vi "Handle Messages.vi"(8 "error in (no error)":errorcluster, 9 "Message Data":variant, 10 "Message":string, 11 "Mock Rig Process In":refnum<class "Mock Process.lvclass">) -> (0 "error out":errorcluster, 3 "Mock Rig Process Out":refnum<class "Mock Process.lvclass">)   [LabVIEW 2020, in "Mock Process.lvclass"]
uses:
  Mock Process.lvclass
  C:/git/astemes-triarc-framework/source/Framework/Process/Process.lvclass
  C:/git/astemes-triarc-framework/source/Framework/Helper Loop/Helper Loop.lvclass
  Mock Process.lvclass/Mock Process.ctl
  Framework/Process/Process.lvclass/Process.ctl
  Framework/Process/Public/Lifecycle/Get Lifecycle State.vi
  Framework/Process/Private/SubVIs/Handle Debug Data.vi
  <vilib>/Utility/error.llb/Clear Errors.vi
  Framework/Logging/Log Debug.vi
  <vilib>/AdvancedString/1D String Array to Delimited String.vi
  <vilib>/Utility/High Resolution Relative Seconds.vi
  Framework/Process/Process.lvclass
  C:/git/astemes-triarc-framework/source/Framework/Logging/Logging.lvclass
  <vilib>/Utility/error.llb/Error Cluster From Error Code.vi
  Framework/Process/Public/Read Name.vi
  <vilib>/ErrorRing/Error Ring.xnode
  Framework/Callback/Callback.lvclass
  Framework/Logging/Logging.lvclass
  Framework/Helper Loop/Helper Loop.lvclass
  C:/git/astemes-triarc-framework/source/Framework/Base/Base.lvclass
  C:/git/astemes-triarc-framework/source/Framework/Configuration File/Configuration File.lvclass
  C:/git/astemes-triarc-framework/source/Framework/Configuration/Configuration.lvclass
  C:/git/astemes-triarc-framework/source/Framework/Error Handler Interface/Error Handler Interface.lvclass
  C:/git/astemes-triarc-framework/source/Framework Test Suite/Mock Process/Mock Process.lvclass
  C:/git/astemes-triarc-framework/source/Framework/Async Handler/Async Handler.lvclass
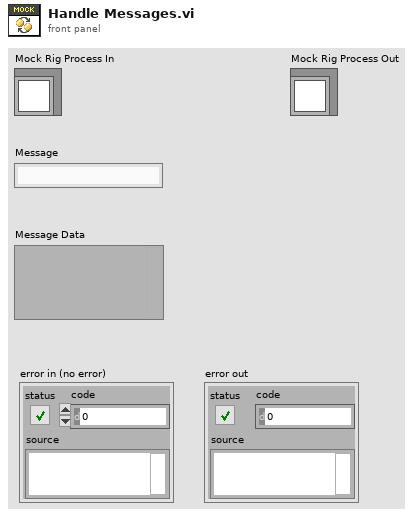
[diagram p1: front panel]
types:
  T1 = cluster{"Message":string, "Message Data":variant}
  T2 = cluster{"Request Message":string, "Request Message Data":variant}
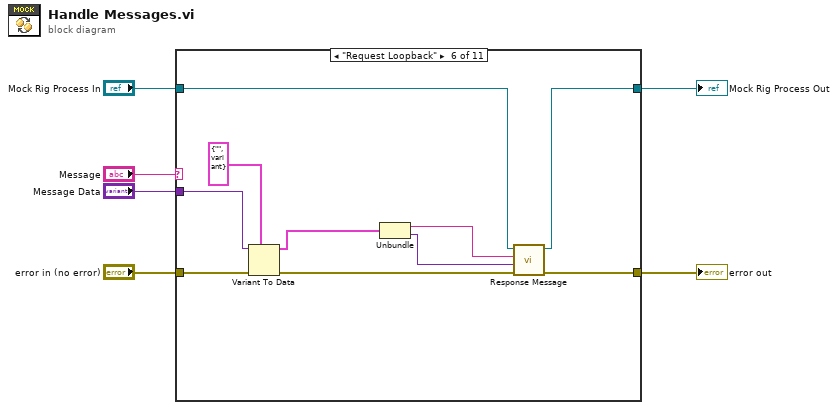
[diagram p0: block diagram]
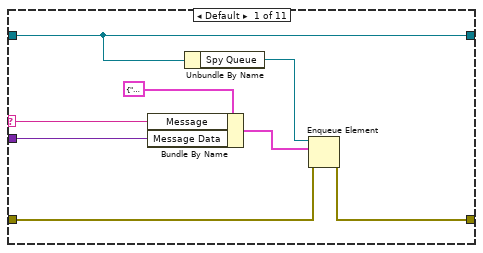
[diagram p2: hidden frame]
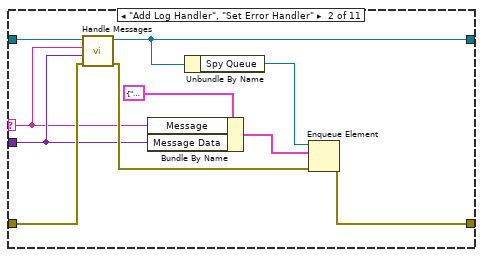
[diagram p3: hidden frame]
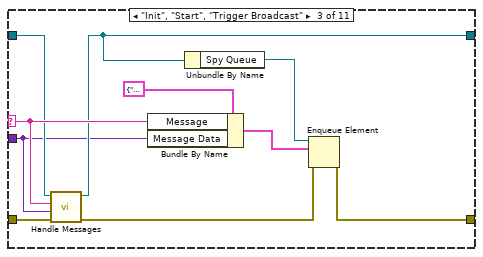
[diagram p4: hidden frame]
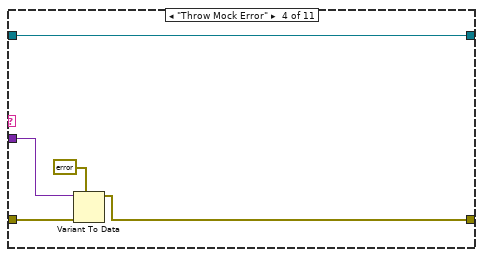
[diagram p5: hidden frame]
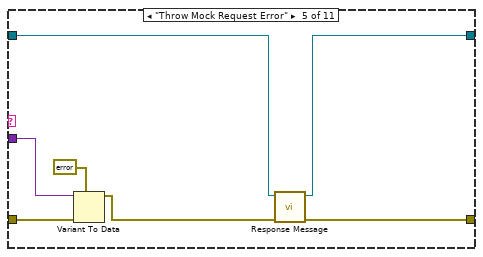
[diagram p6: hidden frame]
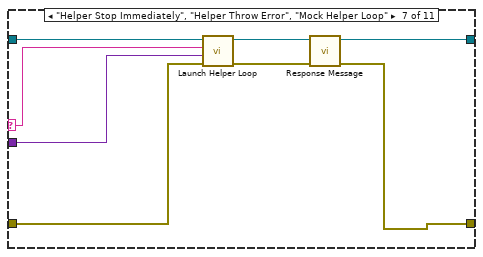
[diagram p7: hidden frame]
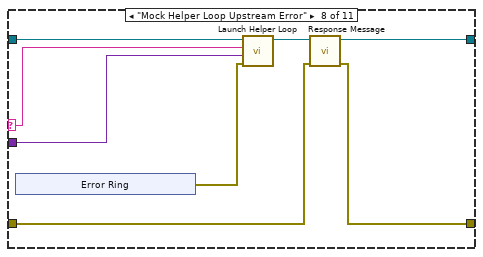
[diagram p8: hidden frame]
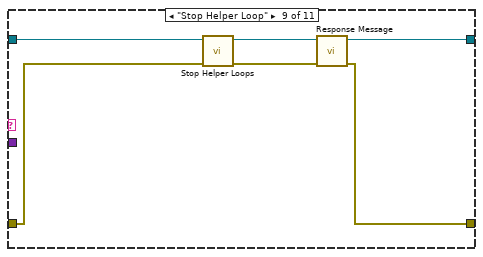
[diagram p9: hidden frame]
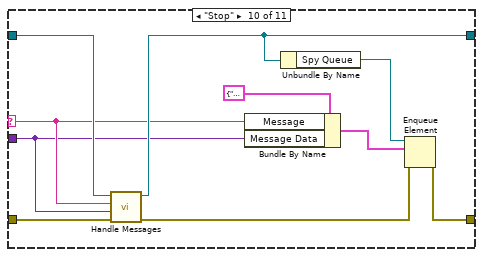
[diagram p10: hidden frame]
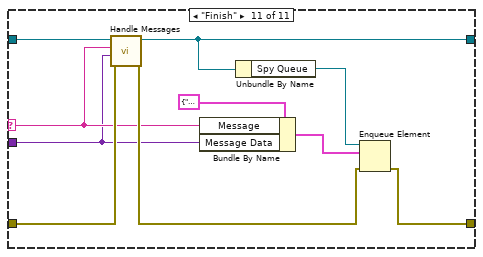
[diagram p11: hidden frame]
diagram:
  n1 = case shown="\"Request Loopback\"" "Message" {
    selector: "Message" -> [w10 w15 w28 _ _ _ w61 w71 _ w84 w94]
    tunnel: [w8 w20 w30 w35 w42 w55 w59 w69 w79 w89 w95] -> w6
    tunnel: [w7 w17 w27 w39 w41 w54 w57 w67 w77 w86 w97] -> w5
    tunnel: "error in (no error)" -> [w9 w21 w31 w38 w46 w56 w63 w66 w81 w87 w101]
    tunnel: "Message Data" -> [w11 w16 w25 w37 w45 w51 w60 w70 _ w83 w93]
    tunnel: "Mock Rig Process In" -> [w7 w18 w26 w39 w40 w53 w64 w72 w82 w85 w102]
    frame Default {
      n2 = Bundle By Name(cluster=T1 {"Message"="", "Message Data"=variant} ("Message Cluster"), "Message"=w10, "Message Data"=w11) -> (w14:T1)
      n3 = Unbundle By Name(w7) -> ("Spy Queue"=w12:refnum<queue>)
      n4 = Enqueue Element(queue=w12, element=w14, error in (no error)=w9) -> (error out=w8:errorcluster)  [unwired: 1 in, 2 out]
    }
    frame "Add Log Handler", "Set Error Handler" {
      n5 = call-parent "Handle Messages.vi"("error in (no error)"=w21, "Message Data"=w16, "Message"=w15, "Process In"=w18) -> ("error out"=w19:errorcluster, "Process Out"=w17:refnum<class "Mock Process.lvclass">)  [unwired: 6 in]
      n6 = Bundle By Name(cluster=T1 {"Message"="", "Message Data"=variant} ("Message Cluster"), "Message"=w15, "Message Data"=w16) -> (w24:T1)
      n7 = Unbundle By Name(w17) -> ("Spy Queue"=w22:refnum<queue>)
      n8 = Enqueue Element(queue=w22, element=w24, error in (no error)=w19) -> (error out=w20:errorcluster)  [unwired: 1 in, 2 out]
    }
    frame "Init", "Start", "Trigger Broadcast" {
      n9 = call-parent "Handle Messages.vi"("error in (no error)"=w31, "Message Data"=w25, "Message"=w28, "Process In"=w26) -> ("error out"=w29:errorcluster, "Process Out"=w27:refnum<class "Mock Process.lvclass">)  [unwired: 6 in]
      n10 = Bundle By Name(cluster=T1 {"Message"="", "Message Data"=variant} ("Message Cluster"), "Message"=w28, "Message Data"=w25) -> (w34:T1)
      n11 = Unbundle By Name(w27) -> ("Spy Queue"=w32:refnum<queue>)
      n12 = Enqueue Element(queue=w32, element=w34, error in (no error)=w29) -> (error out=w30:errorcluster)  [unwired: 1 in, 2 out]
    }
    frame "Throw Mock Error" {
      n13 = Variant To Data(error in=w38, type=errorcluster {"status"=FALSE, "code"=0, "source"=""} ("error out"), Variant=w37) -> (data=w35:errorcluster)  [unwired: 1 out]
    }
    frame "Throw Mock Request Error" {
      n14 = Variant To Data(error in=w46, type=errorcluster {"status"=FALSE, "code"=0, "source"=""} ("error out"), Variant=w45) -> (data=w43:errorcluster)  [unwired: 1 out]
      n15 = call "Response Message.vi"("error in (no error)"=w43, "Process In"=w40) -> ("error out"=w42:errorcluster, "Process Out"=w41:refnum<class "Mock Process.lvclass">)  [unwired: 8 in]
    }
    frame "Request Loopback" {
      n16 = Variant To Data(error in=w56, type=T2 {"Request Message"="", "Request Message Data"=variant} ("output cluster"), Variant=w51) -> (data=w49:T2, error out=w52:errorcluster)
      n17 = Unbundle(w49) -> ("Request Message"=w48:string, "Request Message Data"=w47:variant)
      n18 = call "Response Message.vi"("error in (no error)"=w52, "Response Message Data"=w47, "Response Message"=w48, "Process In"=w53) -> ("error out"=w55:errorcluster, "Process Out"=w54:refnum<class "Mock Process.lvclass">)  [unwired: 6 in]
    }
    frame "Helper Stop Immediately", "Helper Throw Error", "Mock Helper Loop" {
      n19 = call "Launch Helper Loop.vi"("error in (no error)"=w63, "Message Data"=w60, "Message"=w61, "Helper Loop In"=w64) -> ("error out"=w62:errorcluster, "Helper Loop Out"=w58:refnum<class "Mock Process.lvclass">)  [unwired: 6 in]
      n20 = call "Response Message.vi"("error in (no error)"=w62, "Process In"=w58) -> ("error out"=w59:errorcluster, "Process Out"=w57:refnum<class "Mock Process.lvclass">)  [unwired: 8 in]
    }
    frame "Mock Helper Loop Upstream Error" {
      n21 = xnode "Error Ring"() -> ("error out"=w65:errorcluster)
      n22 = call "Launch Helper Loop.vi"("error in (no error)"=w65, "Message Data"=w70, "Message"=w71, "Helper Loop In"=w72) -> ("Helper Loop Out"=w68:refnum<class "Mock Process.lvclass">)  [unwired: 6 in, 1 out]
      n23 = call "Response Message.vi"("error in (no error)"=w66, "Process In"=w68) -> ("error out"=w69:errorcluster, "Process Out"=w67:refnum<class "Mock Process.lvclass">)  [unwired: 8 in]
    }
    frame "Stop Helper Loop" {
      n24 = call "Stop Helper Loops.vi"("error in (no error)"=w81, "Helper Loop In"=w82) -> ("error out"=w80:errorcluster, "Helper Loop Out"=w78:refnum<class "Mock Process.lvclass">)  [unwired: 8 in]
      n25 = call "Response Message.vi"("error in (no error)"=w80, "Process In"=w78) -> ("error out"=w79:errorcluster, "Process Out"=w77:refnum<class "Mock Process.lvclass">)  [unwired: 8 in]
    }
    frame "Stop" {
      n26 = call-parent "Handle Messages.vi"("error in (no error)"=w87, "Message Data"=w83, "Message"=w84, "Process In"=w85) -> ("error out"=w88:errorcluster, "Process Out"=w86:refnum<class "Mock Process.lvclass">)  [unwired: 6 in]
      n27 = Bundle By Name(cluster=T1 {"Message"="", "Message Data"=variant} ("Message Cluster"), "Message"=w84, "Message Data"=w83) -> (w92:T1)
      n28 = Unbundle By Name(w86) -> ("Spy Queue"=w90:refnum<queue>)
      n29 = Enqueue Element(queue=w90, element=w92, error in (no error)=w88) -> (error out=w89:errorcluster)  [unwired: 1 in, 2 out]
    }
    frame "Finish" {
      n30 = call-parent "Handle Messages.vi"("error in (no error)"=w101, "Message Data"=w93, "Message"=w94, "Process In"=w102) -> ("error out"=w96:errorcluster, "Process Out"=w97:refnum<class "Mock Process.lvclass">)  [unwired: 6 in]
      n31 = Bundle By Name(cluster=T1 {"Message"="", "Message Data"=variant} ("Message Cluster"), "Message"=w94, "Message Data"=w93) -> (w100:T1)
      n32 = Unbundle By Name(w97) -> ("Spy Queue"=w99:refnum<queue>)
      n33 = Enqueue Element(queue=w99, element=w100, error in (no error)=w96) -> (error out=w95:errorcluster)  [unwired: 1 in, 2 out]
    }
  }
  "error out" <- w6
  "Mock Rig Process Out" <- w5
